vi "Init.vi"(8 "error in (no error)":errorcluster, 11 "Tool in":refnum<class "MockTool.lvclass">) -> (0 "error out":errorcluster, 3 "Tool out":refnum<class "MockTool.lvclass">)   [LabVIEW 2017, in "MockTool.lvclass"]
uses:
  MockTool.lvclass
  C:/Users/Jan/Projects/opentool-labview/Server/ITool/ITool.lvclass
  Server/ITool/ITool.lvclass
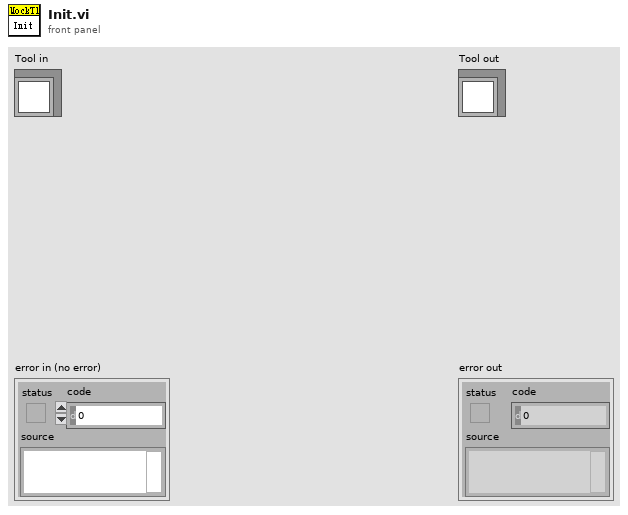
[diagram p1: front panel]
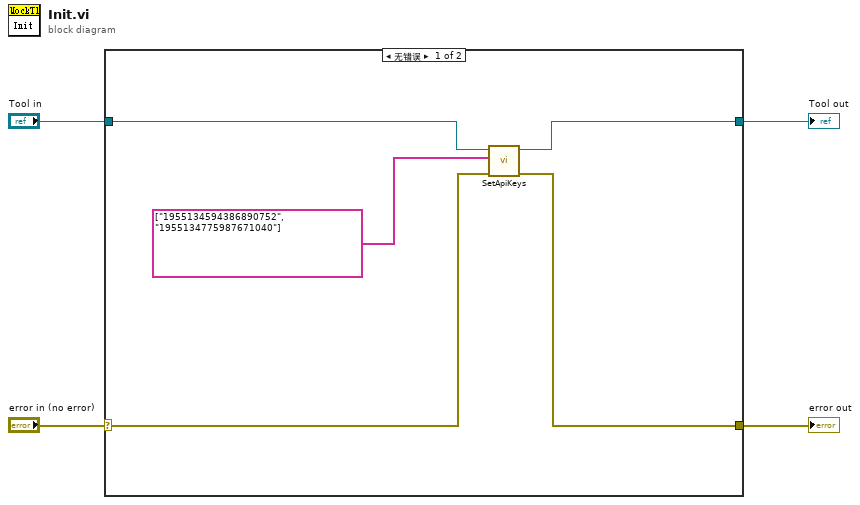
[diagram p0: block diagram]
diagram:
  n1 = case shown="无错误" "error in (no error)" {
    selector: "error in (no error)" -> [w7 w10]
    tunnel: [w6 w10] -> w3
    tunnel: "Tool in" -> [w9 w11]
    tunnel: [w8 w11] -> w1
    frame No Error {
      n2 = call "SetApiKeys.vi"("error in (no error)"=w7, "ApiKeys"=string[] ["1955134594386890752", "1955134775987671040"], "ITool in"=w9) -> ("error out"=w6:errorcluster, "ITool out"=w8:refnum<class "MockTool.lvclass">)  [unwired: 7 in]
    }
    frame Error {
    }
  }
  "Tool out" <- w1
  "error out" <- w3
